vi "change tag type.vi"(7 "owner ID":string, 8 "error in":errorcluster, 9 "new data type":T1, 10 "tag name":string, 11 "engine configuration in":refnum<class "engine configuration.lvclass">) -> (0 "error out":errorcluster, 3 "engine configuration out":refnum<class "engine configuration.lvclass">)   [LabVIEW 2014, in "engine configuration.lvclass"]
doc: "This function is used to change the data type of a tag. Changing a tag's data type removes any channel mappings associated with that tag."
uses:
  engine configuration.lvclass
  <vilib>/NI/Tag Bus/tag/Data Type.ctl
  <vilib>/NI/Tag Bus/tag/tag descriptor.lvclass
  <vilib>/NI/Tag Bus/tag/tag descriptor.lvclass/tag descriptor.ctl
  engine configuration.lvclass/engine configuration.ctl
  module channel pairings.ctl
  <vilib>/NI/Tag Bus/tag/write tag name.vi
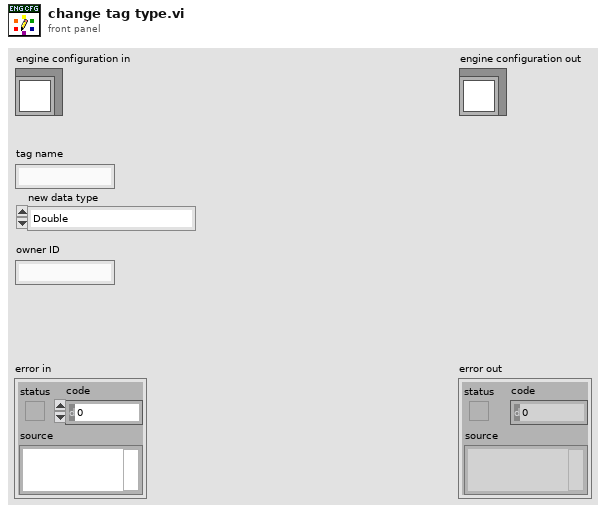
[diagram p1: front panel]
types:
  T1 = typedef "tag bus.lvlib/tag descriptor.lvclass/Data Type.ctl" = enum16{"Double", "Single", "I64", "I32", "I16", "I8", "U64", "U32", "U16", "U8", "Boolean", "String", "Array of Double", "Array of Single", "Array of I64", "Array of I32", "Array of I16", "Array of I8", "Array of U64", "Array of U32", "Array of U16", "Array of U8", "Array of Boolean", "Array of String"}
  T2 = typedef "engine configuration.lvclass/module channel pairings.ctl" = cluster{"modules":string[], "channels":string[]}
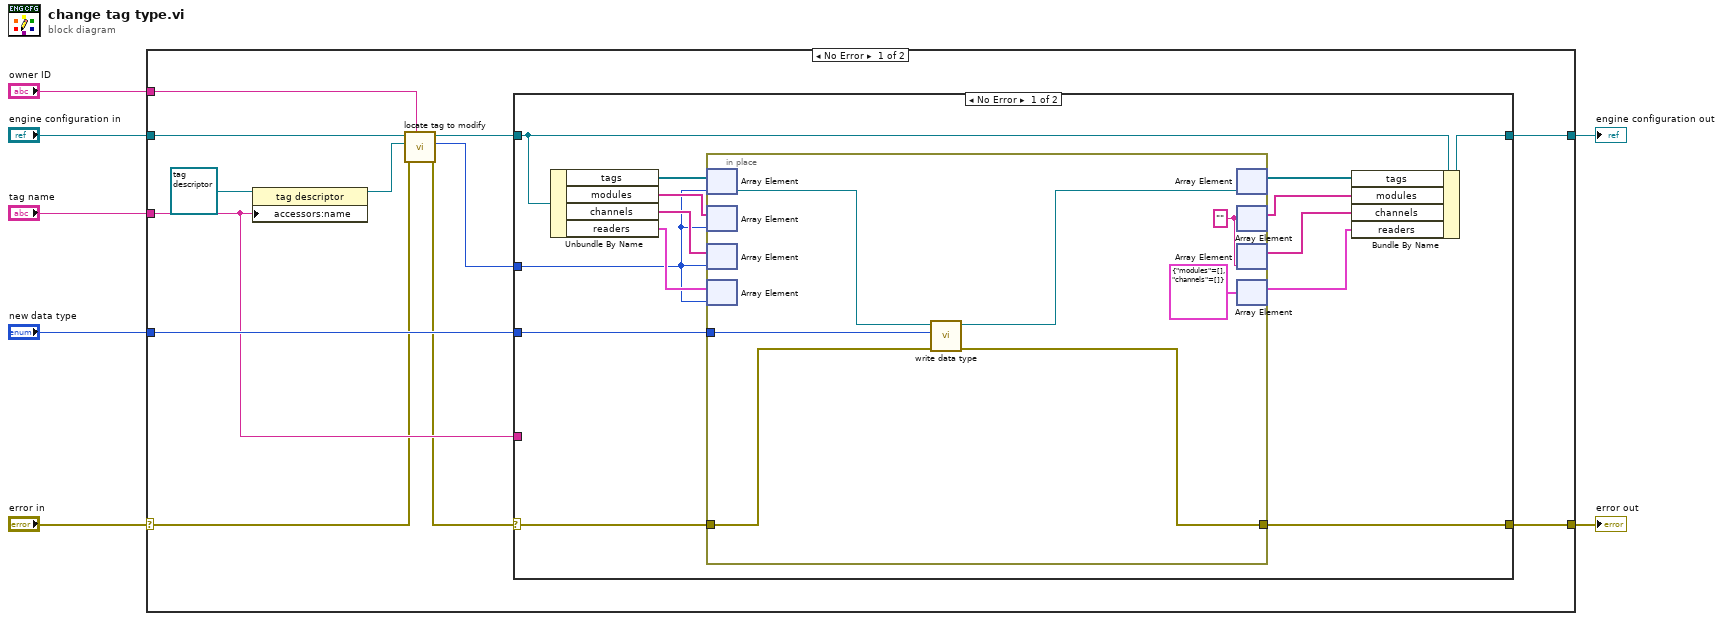
[diagram p0: block diagram]
diagram:
  n1 = case shown="No Error" "error in" {
    selector: "error in" -> [w10 w44]
    tunnel: [w17 w44] -> w6
    tunnel: [w18 w43] -> w4
    tunnel: "engine configuration in" -> [w14 w43]
    tunnel: "tag name" -> [w15 _]
    tunnel: "new data type" -> [w16 _]
    tunnel: "owner ID" -> [w11 _]
    frame No Error {
      n2 = property class="tag descriptor"(reference=refnum<class "tag descriptor.lvclass"> refnum ("tag descriptor"), "accessors:name"=w15) -> (reference out=w12:refnum<class "tag descriptor.lvclass">)  [unwired: 1 in, 1 out]
      n3 = call "locate tag to modify.vi"("owner ID"=w11, "error in"=w10, "tag descriptor"=w12, "engine configuration in"=w14) -> ("error out"=w9:errorcluster, "index"=w8:i32, "engine configuration out"=w13:refnum<class "engine configuration.lvclass">)  [unwired: 5 in]
      n4 = case shown="No Error" w9 {
        selector: w9 -> [w21 w41]
        tunnel: w13 -> [w32 w42]
        tunnel: [w33 w42] -> w18
        tunnel: [w20 w41] -> w17
        tunnel: w16 -> [w22 _]
        tunnel: w15 -> [_ _]
        tunnel: w8 -> [w23 _]
        frame No Error {
          n5 = Unbundle By Name(w32) -> ("tags"=w31:refnum<class "tag descriptor.lvclass">[], "modules"=w26:string[], "channels"=w25:string[], "readers"=w24:T2[])
          n6 = in-place {
            in-place-border: w22 -> [w39]
            in-place-border: w21 -> [w37]
            in-place-border: [w36] -> w20
            w35 = "" ("element")
            n7 = in-place-array #1(w31, w23) -> (w40:refnum<class "tag descriptor.lvclass">)
            n8 = in-place-array #2(w26, w23) -> ()  [unwired: 1 out]
            n9 = in-place-array #3(w25, w23) -> ()  [unwired: 1 out]
            n10 = in-place-array #4(w24, w23) -> ()  [unwired: 1 out]
            n11 = call <vilib>:"write data type.vi"("error in"=w37, "data type"=w39, "system tag in"=w40) -> ("error out"=w36:errorcluster, "system tag out"=w38:refnum<class "tag descriptor.lvclass">)  [unwired: 7 in]
            n12 = in-place-array #1(w38) -> (w30:refnum<class "tag descriptor.lvclass">[])  [unwired: 1 out]
            n13 = in-place-array #2(w35) -> (w29:string[])  [unwired: 1 out]
            n14 = in-place-array #3(w35) -> (w28:string[])  [unwired: 1 out]
            n15 = in-place-array #4(T2 {"modules"=[], "channels"=[]} ("element")) -> (w27:T2[])  [unwired: 1 out]
          }
          n16 = Bundle By Name(cluster=w32, "tags"=w30, "modules"=w29, "channels"=w28, "readers"=w27) -> (w33:refnum<class "engine configuration.lvclass">)
        }
        frame Error {
        }
      }
    }
    frame Error {
    }
  }
  "error out" <- w6
  "engine configuration out" <- w4
